vi "PicoScope5000aExampleBlockMSO.vi"() -> ()   [LabVIEW 2010]
uses:
  shared/PicoBuffers.ctl
  <vilib>/Waveform/DWDTOps.llb/DWDT Analog to Digital.vi
  PicoScope5000aLib/PicoScope5000aAnalogChannelSettings.ctl
  PicoScope5000aLib/PicoScope5000aDigitalChannelSettings.ctl
  shared/Buffer and Transfer Settings.ctl
  shared/Acquisition Settings.ctl
panel:
  in  "Channel B Settings":T1={"Enabled"=FALSE, "Coupling"=1, "Range"=6, "Analogue Offset"=0.0, "Bandwidth Limit"=0} {"Bandwidth Limit" items=["Full", "20MHz"]; "Range" items=["10 mV", "20 mV", "50 mV", "100 mV", "200 mV", "500 mV", "1 V", "2 V", "5 V", "10 V", "20 V"]; "Coupling" items=["AC", "DC"]}
  out "overflow":i16 format="%010b"
  in  "Apply Settings":bool
  in  "Port 0 Settings":T2={"Enabled"=FALSE, "Logic Level"=9830} {"Logic Level" items=["1.5V TTL"=9830, "2.5V CMOS"=16383]}
  in  "Channel A Settings":T1={"Enabled"=TRUE, "Coupling"=1, "Range"=6, "Analogue Offset"=0.0, "Bandwidth Limit"=0} {"Bandwidth Limit" items=["Full", "20MHz"]; "Range" items=["10 mV", "20 mV", "50 mV", "100 mV", "200 mV", "500 mV", "1 V", "2 V", "5 V", "10 V", "20 V"]; "Coupling" items=["AC", "DC"]}
  in  "Trigger Settings":T3={"Trigger Enabled"=FALSE, "Trigger Source"=enum."Channel A", "Trigger Threshold (volts)"=0.0, "Trigger Direction"=2, "Trigger Delay (samples)"=0, "Auto Trigger Time (ms)"=1000} {"Trigger Direction" items=["Rising"=2, "Falling"=3]}
  out "USB 3.0 device on non-USB 3.0 Port":bool=TRUE
  out "USB Powered":bool=TRUE
  out "Device Info":T4={"Driver Version"="2.1.104.3324", "USB Version"="2.0", "Hardware"="1", "Variant"="5244A", "Batch and Serial"="CQ178/007", "Cal Date"="11Jun13", "Kernel Version"="1.0", "Digital HW Version"="1", "Analogue HW Version"="1", "MSO"=FALSE, "Number of channels"=2}
  out "error out":errorcluster
  in  "Data file":path=path "PicoScope5000aExampleBlock ChA Data"
  in  "Buffer and Transfer Settings":T5={"startIndex"=0, "Samples"=5000000, "Down Sample Ratio"=1, "Down-Sample Mode"=0} {"Down-Sample Mode" items=["RAW none"=2147483648, "None"=0, "Aggregate"=1, "Decimate"=2, "Average"=4]; "Down Sample Ratio" step=1; "Samples" format="%_6p"}
  in  "Acquisition Settings":T6={"preTriggerSamples"=0, "postTriggerSamples"=5000000, "timebase"=5} {"postTriggerSamples" format="%_6p"; "preTriggerSamples" format="%_6p"}
  out "Properties Panel":T7={"Sample Frequency"=41666668.0, "Sample Rate"=2.4000000209412065e-08, "Max Samples Available"=26843008, "Number of Samples"=0, "Total Capture Time (sec) "=0.0, "Max Total Capture Time Available (sec)"=0.6442322134971619} {"Max Total Capture Time Available (sec)" format="%.3p"; "Sample Frequency" format="%.6p"; "Sample Rate" format="%.3p"; "Max Samples Available" format="%_6p"; "Total Capture Time (sec)" format="%.3p"}
  out "Port 0":digitalwaveform(graph)={"t0"=timestamp(0 s since 1904-01-01), "dt"=8e-09, "Y"={"transitions"=[], "data"=[]}}
  in  "stop":bool
  out "Analog Channels":cluster{i32, sgl, "Data":dbl[]}[](graph)
  in  "Resolution":u32(ring) items=["8-bit"=0, "12-bit"=1, "14-bit"=2, "15-bit"=3, "16-bit"=4, "10-bit"=10]
  in  "Serial Number":string
  in  "Use Serial Number":bool
  in  "error in (no error)":errorcluster
  # "Bit 0 = ChA"
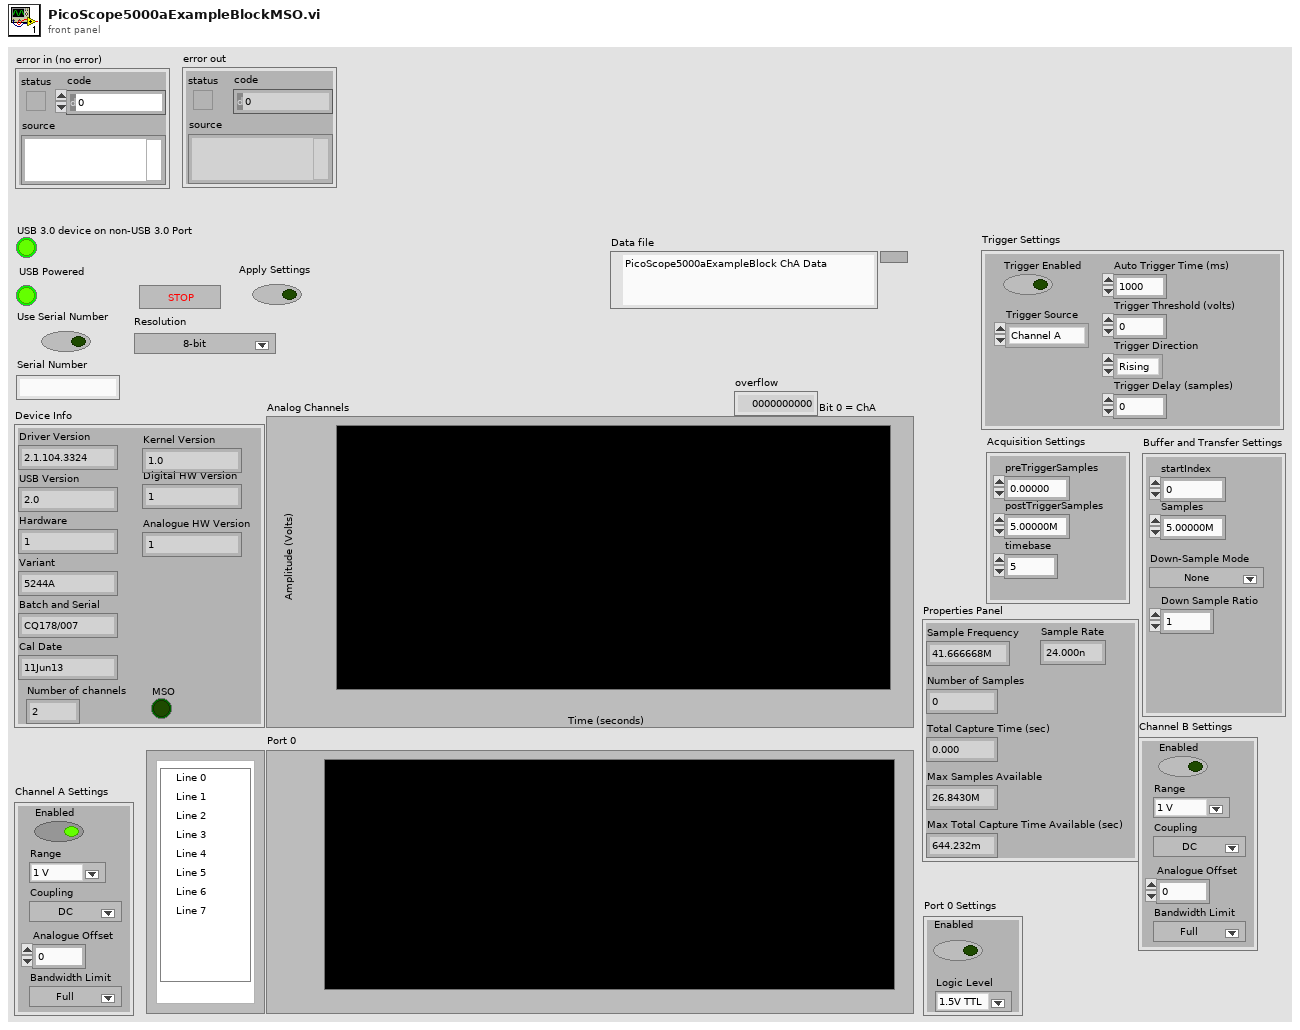
[diagram p1: front panel]
types:
  T1 = typedef "PicoScope5000aAnalogChannelSettings.ctl" = cluster{"Enabled":bool, "Coupling":i16, "Range":u16, "Analogue Offset":sgl, "Bandwidth Limit":u32}
  T2 = typedef "PicoScope5000aDigitalChannelSettings.ctl" = cluster{"Enabled":bool, "Logic Level":i16}
  T3 = cluster{"Trigger Enabled":bool, "Trigger Source":enum16{"Channel A", "Channel B", "Channel C", "Channel D", "Ext."}, "Trigger Threshold (volts)":dbl, "Trigger Direction":u16, "Trigger Delay (samples)":u32, "Auto Trigger Time (ms)":i16}
  T4 = cluster{"Driver Version":string, "USB Version":string, "Hardware":string, "Variant":string, "Batch and Serial":string, "Cal Date":string, "Kernel Version":string, "Digital HW Version":string, "Analogue HW Version":string, "MSO":bool, "Number of channels":i16}
  T5 = typedef "Buffer and Transfer Settings.ctl" = cluster{"startIndex":u64, "Samples":u64, "Down Sample Ratio":u64, "Down-Sample Mode":u32}
  T6 = typedef "Acquisition Settings.ctl" = cluster{"preTriggerSamples":u64, "postTriggerSamples":u64, "timebase":u32}
  T7 = cluster{"Sample Frequency":dbl, "Sample Rate":dbl, "Max Samples Available":u64, "Number of Samples":u64, "Total Capture Time (sec) ":dbl, "Max Total Capture Time Available (sec)":dbl}
  T8 = typedef "PicoBuffers.ctl" = cluster{"Max Buffer Pointers":u64[][][], "Min Buffer Pointers":u64[][][], "StreamingDataInfo":cluster{"Channel":u32, "Down-Sample Mode":u32, "PICO_DATA_TYPE":enum32{"PICO_INT8_T", "PICO_INT16_T", "PICO_INT32_T", "PICO_UINT32_T", "PICO_INT64_T", ""}, "Samples":i32, "bufferIndex":u64, "startIndex":i32, "overflow":i16}[][]}
  T9 = enum16{"open", "open or create", "create or replace", "create", "open (read-only)"}
  T10 = cluster{"Sample Frequency":sgl, "Sample Rate":sgl, "Max Samples Available":i32, "Number of Samples":u32, "Total Capture Time (sec) ":sgl, "Max Total Capture Time Available (sec)":sgl}
  T11 = cluster{"Channel A Buffer":i16[], "Channel B Buffer":i16[], "Channel C Buffer":i16[], "Channel D Buffer":i16[], "Channel E Buffer":i16[], "Channel F Buffer":i16[], "Channel G Buffer":i16[], "Channel H Buffer":i16[], "Port 0 Buffer":i16[], "Port 1 Buffer":i16[]}[]
  T12 = cluster{"Channel A Buffer":i16[], "Channel B Buffer":i16[], "Channel C Buffer":i16[], "Channel D Buffer":i16[], "Channel E Buffer":i16[], "Channel F Buffer":i16[], "Channel G Buffer":i16[], "Channel H Buffer":i16[], "Port 0 Buffer":i16[], "Port 1 Buffer":i16[]}
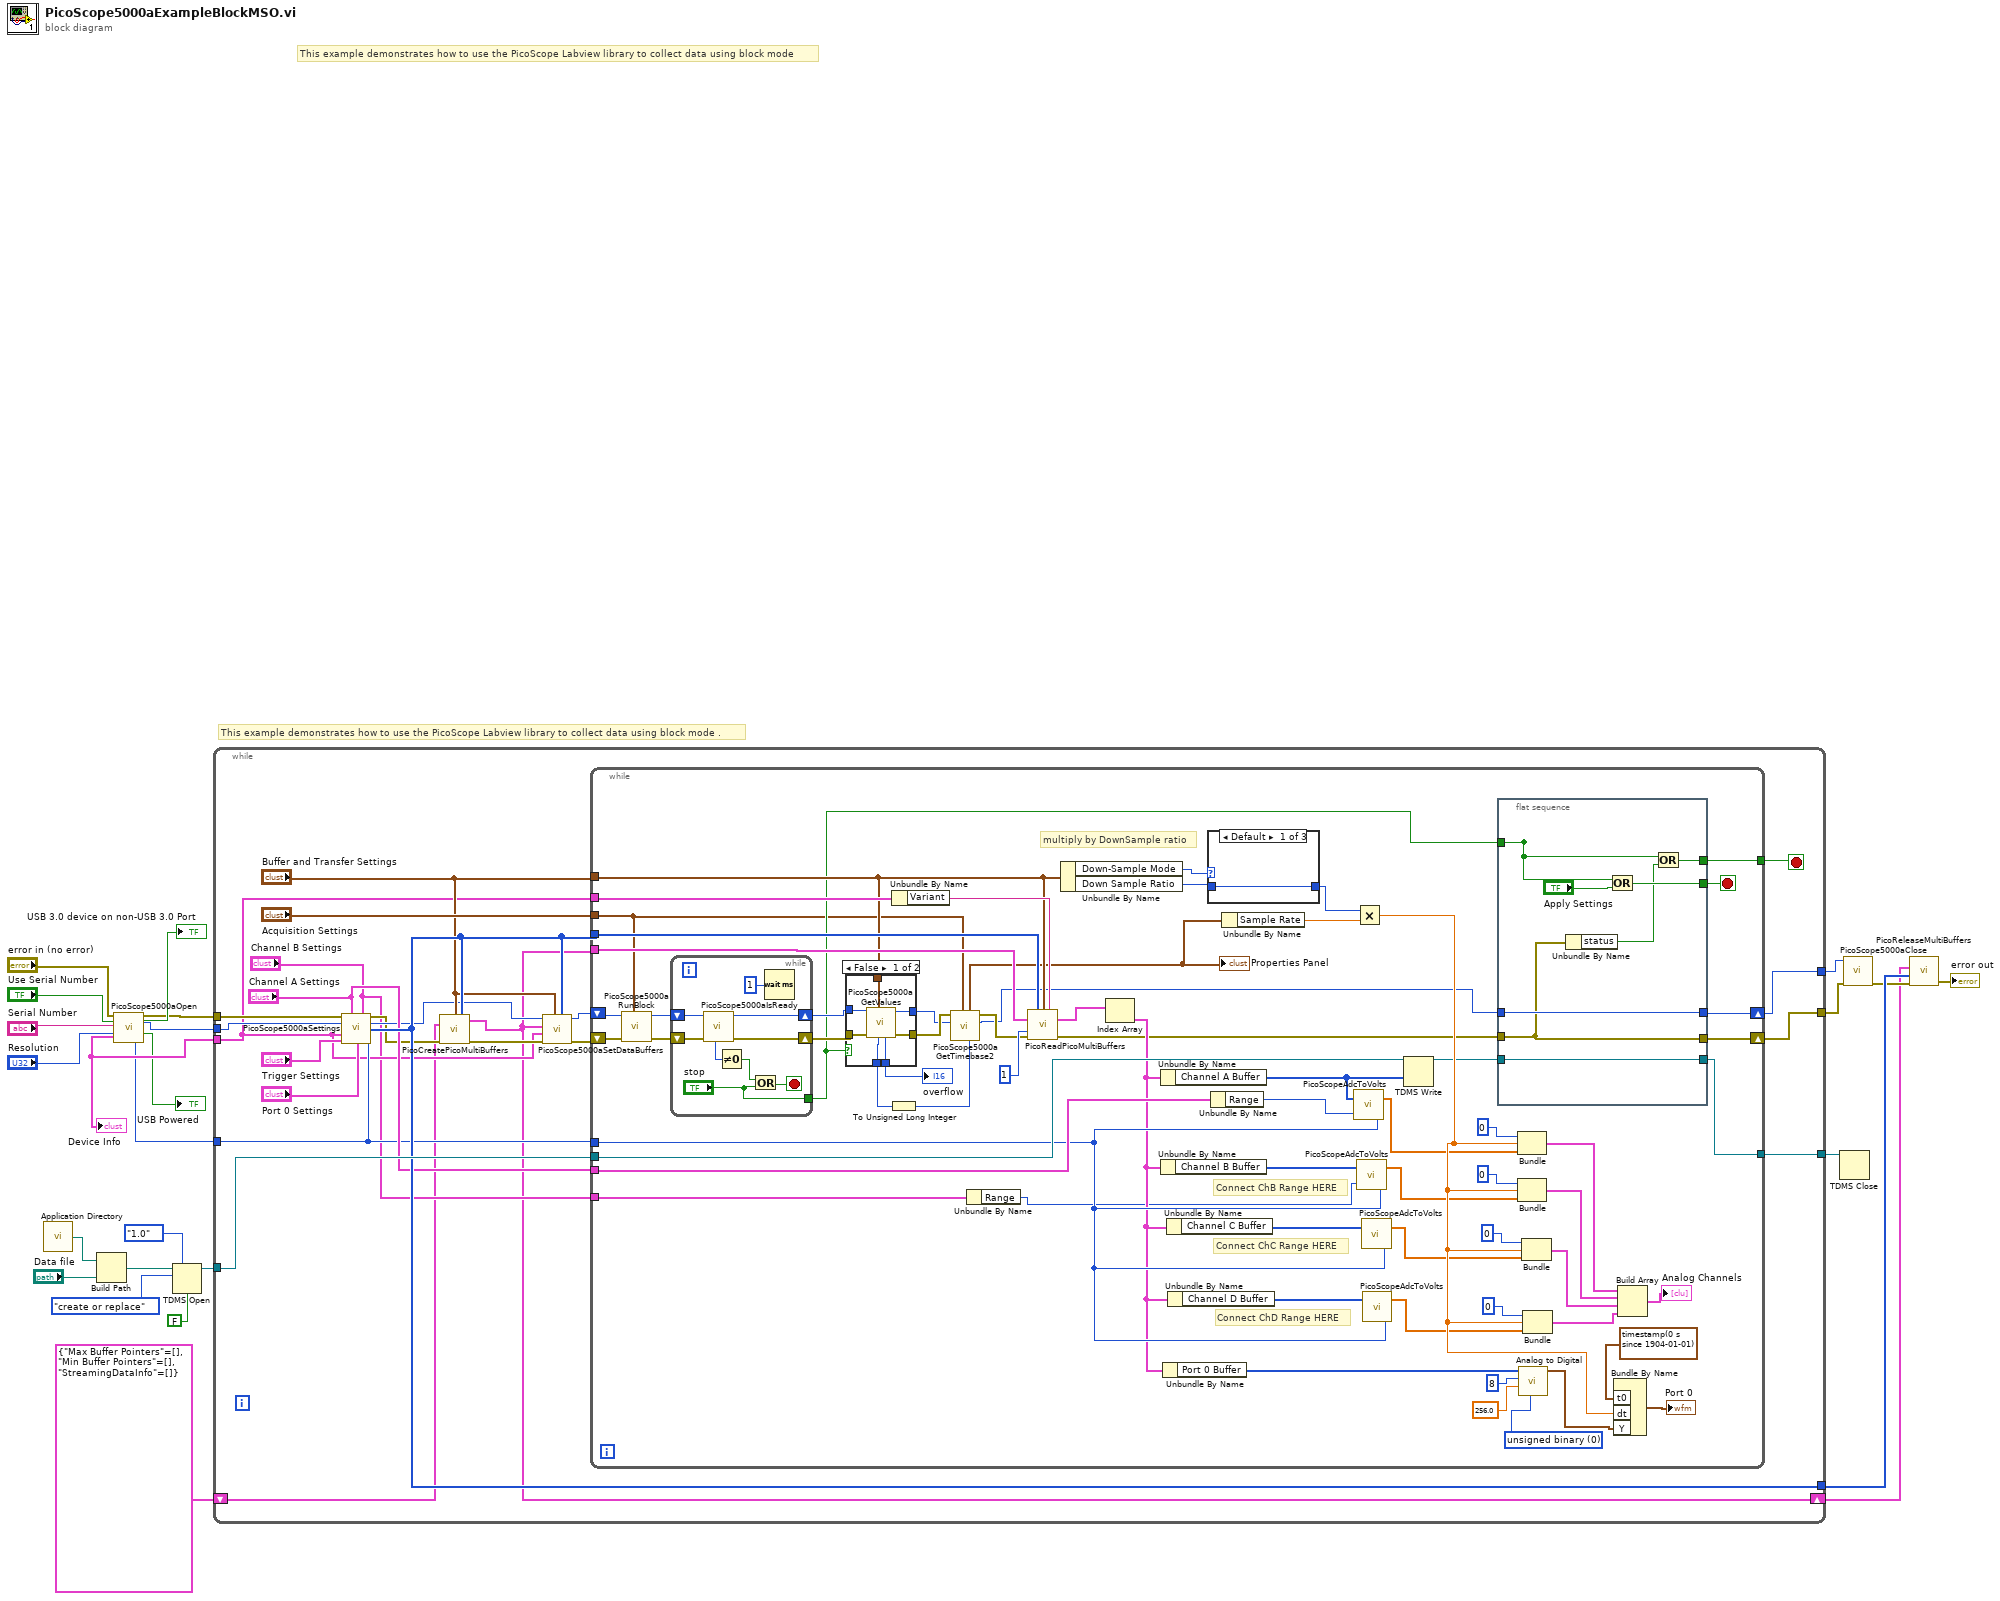
[diagram p0: block diagram]
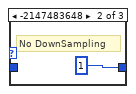
[diagram p3: hidden frame]
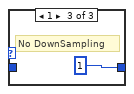
[diagram p4: hidden frame]
diagram:
  # "This example demonstrates how to use the PicoScope Labview library to collect data using block mode ."
  # "This example demonstrates how to use the PicoScope Labview library to collect data using block mode"
  n1 = call <vilib>:"Application Directory.vi"() -> ("Application Directory"=w18:path)
  n2 = Build Path(base path=w18, name or relative path="Data file") -> (appended path=w19:path)
  n3 = call "PicoScope5000aOpen.vi"("error in (no error)"="error in (no error)", "Serial Number"="Serial Number", "Use Serial Number"="Use Serial Number", "Resolution"="Resolution") -> ("USB 3.0 device on non-USB 3.0 Port"=→"USB 3.0 device on non-USB 3.0 Port":bool, "error out"=w6:errorcluster, "handle"=w25:i16, "USB Powered"=→"USB Powered":bool, "Device Info"=w10:T4, "Max ADC value"=w9:i16)  [unwired: 6 in]
  "Device Info" <- w10
  n4 = TDMS Open(6:FALSE ("disable buffering? (T)"), 7:enum16{"1.0", "2.0"}."1.0" ("file format version (2.0)"), 10:T9."create or replace" ("operation (0:open)"), 11:w19) -> (3:w16:refnum<k34>)  [unwired: 2 in, 1 out]
  n5 = while {
    tunnel: w25 -> [w46]
    tunnel: w9 -> [w39]
    tunnel: [w43] -> w24
    tunnel: [w37] -> w17
    tunnel: w16 -> [w47]
    tunnel: w10 -> [w29]
    tunnel: w6 -> [w45]
    tunnel: [w38] -> w4
    tunnel: [w35] -> w5
    shift-right: [w26] -> w1
    shift-left: T8 {"Max Buffer Pointers"=[], "Min Buffer Pointers"=[], "StreamingDataInfo"=[]} ("Data Pointers") -> [w27]
    stop <- w36 stop-if-true
    n6 = call "PicoScope5000aSettings.vi"("error in"=w45, "Channel A Settings"="Channel A Settings", "Port 0 Settings"="Port 0 Settings", "Channel B Settings"="Channel B Settings", "handle in"=w46, "Device Info"=w29, "Trigger Settings"="Trigger Settings", "Max ADC value"=w39) -> ("error out"=w30:errorcluster, "handle out"=w31:i16, "enabled array"=w43:i16[])  [unwired: 5 in]
    n7 = call "PicoCreatePicoMultiBuffers.vi"("Buffer and Transfer Settings"="Buffer and Transfer Settings", "enabled array"=w43, "Data Pointers In"=w27, "error in (no error)"=w30) -> ("Data Pointers"=w26:T8, "error out"=w48:errorcluster)  [unwired: 10 in]
    n8 = call "PicoScope5000aSetDataBuffers.vi"("enabled array"=w43, "Buffer and Transfer Settings"="Buffer and Transfer Settings", "error in (no error)"=w48, "Device Info"=w29, "Data Pointers In"=w26, "handle in"=w31) -> ("error out"=w34:errorcluster, "handle out"=w33:i16)  [unwired: 4 in]
    n9 = while {
      tunnel: w26 -> [w114]
      tunnel: "Buffer and Transfer Settings" -> [w61]
      tunnel: w43 -> [w105]
      tunnel: "Channel A Settings" -> [w104]
      tunnel: "Acquisition Settings" -> [w53]
      tunnel: w39 -> [w103]
      tunnel: w29 -> [w100]
      tunnel: [w68] -> w36
      shift-right: [w72] -> w38
      shift-left: w34 -> [w62]
      shift-right: [w66] -> w35
      shift-left: w33 -> [w63]
      tunnel: w47 -> [w113]
      tunnel: [w70] -> w37
      tunnel: "Channel B Settings" -> [w49]
      stop <- w67 stop-if-true
      w89 = u16 0 items=["unsigned binary", "offset binary", "2's complement"] ("data format (offset binary)")
      # "Connect ChB Range HERE"
      # "Connect ChD Range HERE"
      # "Connect ChC Range HERE"
      # "multiply by DownSample ratio"
      n10 = call "PicoScope5000aRunBlock.vi"("Acquisition Settings"=w53, "error in (no error)"=w62, "handle in"=w63) -> ("error out"=w107:errorcluster, "handle out"=w106:i16)  [unwired: 5 in, 2 out]
      n11 = while {
        shift-right: [w139] -> w64
        shift-left: w107 -> [w140]
        shift-right: [w138] -> w65
        shift-left: w106 -> [w137]
        tunnel: ["stop"] -> w60
        stop <- w134 stop-if-true
        n12 = call "PicoScope5000aIsReady.vi"("error in (no error)"=w140, "handle in"=w137) -> ("error out"=w139:errorcluster, "handle out"=w138:i16, "ready"=w136:i16)  [unwired: 7 in]
        n13 = Not Equal To 0?(x=w136) -> (x != 0?=w135:bool)
        n14 = Or(x=w135, y="stop") -> (x .or. y?=w134:bool)
        n15 = Wait (ms)(milliseconds to wait=u32 1) -> ()  [unwired: 1 out]
      }
      n16 = case shown="False" w60 {
        tunnel: w64 -> [w121 w122]
        tunnel: w65 -> [w120 w123]
        tunnel: [w119 w123] -> w57
        tunnel: [w118 w122] -> w58
        tunnel: w61 -> [w117 _]
        tunnel: [w116 _] -> w59
        tunnel: [w115 _] -> w52
        frame False {
          n17 = call "PicoScope5000aGetValues.vi"("Buffer and Transfer Settings"=w117, "error in (no error)"=w121, "handle in"=w120) -> ("error out"=w118:errorcluster, "handle out"=w119:i16, "overflow"=w116:i16, "noOfSamples"=w115:u64)  [unwired: 5 in]
        }
        frame True {
        }
      }
      "overflow" <- w59
      n18 = To Unsigned Long Integer(number=w52) -> (unsigned 32bit integer=w51:u32)
      n19 = Unbundle By Name(w100) -> ("Variant"=w101:string)
      n20 = call "PicoScope5000aGetTimebase2.vi"("Number of Samples"=w51, "Acquisition Settings"=w53, "handle in"=w57, "error in (no error)"=w58) -> ("handle out"=w55:i16, "error out"=w56:errorcluster, "Properties Panel"=w54:T10)  [unwired: 5 in]
      "Properties Panel" <- w54
      n21 = Unbundle By Name(w49) -> ("Range"=w50:u16)
      n22 = call "PicoReadPicoMultiBuffers.vi"("enabled array"=w105, "Buffer and Transfer Settings"=w61, "Variant"=w101, "Data Pointers"=w114, "No of Buffers"=1, "error in (no error)"=w56) -> ("MultiBuffers (Max or non-aggregated)"=w112:T11, "error out"=w69:errorcluster)  [unwired: 7 in, 1 out]
      n23 = Unbundle By Name(w61) -> ("Down-Sample Mode"=w110:u32, "Down Sample Ratio"=w111:u64)
      n24 = Index Array(array=w112) -> (element=w73:T12)  [unwired: 1 in]
      n25 = Unbundle By Name(w73) -> ("Channel A Buffer"=w82:i16[])
      n26 = Unbundle By Name(w73) -> ("Channel B Buffer"=w95:i16[])
      n27 = Unbundle By Name(w73) -> ("Port 0 Buffer"=w87:i16[])
      n28 = Unbundle By Name(w73) -> ("Channel C Buffer"=w80:i16[])
      n29 = Unbundle By Name(w73) -> ("Channel D Buffer"=w76:i16[])
      n30 = case shown="Default" w110 {
        tunnel: [w141 u64 1 ("Down Sample Ratio") u64 1 ("Down Sample Ratio")] -> w108
        tunnel: w111 -> [w141 _ _]
        frame Default {
        }
        frame -2147483648 {
          # "No DownSampling"
        }
        frame 1 {
          # "No DownSampling"
        }
      }
      n31 = Unbundle By Name(w104) -> ("Range"=w97:u16)
      n32 = Unbundle By Name(w54) -> ("Sample Rate"=w102:sgl)
      n33 = call "PicoScopeAdcToVolts.vi"("Max_adc"=w103, "Range Index"=w97, "Data"=w82) -> ("Data"=w83:dbl[])
      n34 = Multiply(x=w108, y=w102) -> (x*y=w109:sgl)
      n35 = call "PicoScopeAdcToVolts.vi"("Max_adc"=w103, "Range Index"=w50, "Data"=w95) -> ("Data"=w94:dbl[])
      n36 = call "PicoScopeAdcToVolts.vi"("Max_adc"=w103, "Data"=w80) -> ("Data"=w79:dbl[])  [unwired: 1 in]
      n37 = call "PicoScopeAdcToVolts.vi"("Max_adc"=w103, "Data"=w76) -> ("Data"=w75:dbl[])  [unwired: 1 in]
      n38 = TDMS Write(0:w113, 9:w82) -> (4:w71:refnum<k34>)  [unwired: 4 in, 3 out]
      n39 = flat-sequence {
        tunnel: [w131] -> w67
        tunnel: [w124] -> _
        tunnel: [w128] -> w68
        tunnel: w55 -> [w127]
        tunnel: [w127] -> w66
        tunnel: w69 -> [w126]
        tunnel: [w126] -> w72
        tunnel: [w125] -> w70
        tunnel: w71 -> [w125]
        tunnel: w60 -> [w124]
        frame #0 {
          n40 = Unbundle By Name(w126) -> ("status"=w129:bool)
          n41 = Or(x=w124, y="Apply Settings") -> (x .or. y?=w131:bool)
          n42 = Or(x=w124, y=w129) -> (x .or. y?=w128:bool)
        }
      }
      n43 = Bundle(0, w109, "Data"=w83) -> (w93:cluster{i32, sgl, "Data":dbl[]})  [unwired: 1 in]
      n44 = Bundle(0, w109, "Data"=w94) -> (w92:cluster{i32, sgl, "Data":dbl[]})  [unwired: 1 in]
      n45 = call-poly <vilib>:"Analog to Digital.vi"("data format (offset binary)"=w89, "full-scale range (pk-pk)"=256.0, "resolution (16 bit)"=8, "analog waveform"=w87) -> ("digital waveform"=w84:digitalwaveform)  [unwired: 4 in, 3 out]
      n46 = Bundle(0, w109, "Data"=w79) -> (w78:cluster{i32, sgl, "Data":dbl[]})  [unwired: 1 in]
      n47 = Bundle(0, w109, "Data"=w75) -> (w74:cluster{i32, sgl, "Data":dbl[]})  [unwired: 1 in]
      n48 = Bundle By Name("t0"=timestamp(0 s since 1904-01-01), "dt"=w109, "Y"=w84) -> (→"Port 0":digitalwaveform)  [unwired: 1 in]
      n49 = Build Array(w93, w92, w78, w74) -> (→"Analog Channels":cluster{i32, sgl, "Data":dbl[]}[])
    }
  }
  n50 = TDMS Close(11:w17) -> ()  [unwired: 1 in, 2 out]
  n51 = call "PicoScope5000aClose.vi"("error in (no error)"=w4, "handle in"=w5) -> ("error out"=w3:errorcluster)  [unwired: 8 in, 1 out]
  n52 = call "PicoReleaseMultiBuffers.vi"("error in (no error)"=w3, "Enabled array"=w24, "Data Pointers"=w1) -> ("error out"=→"error out":errorcluster)  [unwired: 7 in, 1 out]
